vi "FRC Display Status Dialog.vi"(8 "error in":errorcluster, 9 "Numeric":u8, 10 "Text":string, 11 "Mode":T1(ring)) -> (0 "error out":errorcluster)   [LabVIEW 2027]
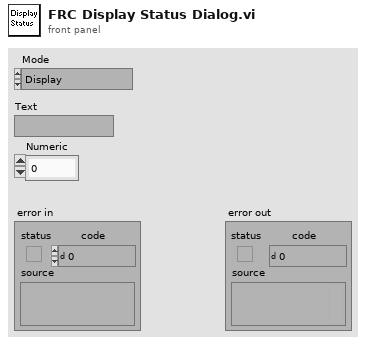
[diagram p1: front panel]
types:
  T1 = enum16{"Display", "Configure", "Hide Dialog", "Discard Ref"}
  T2 = enum32{"Invalid", "Standard", "Closed", "Hidden", "Minimized", "Maximized"}
  T3 = cluster{"Quit":bool, "Message":string, "Numeric":u8}
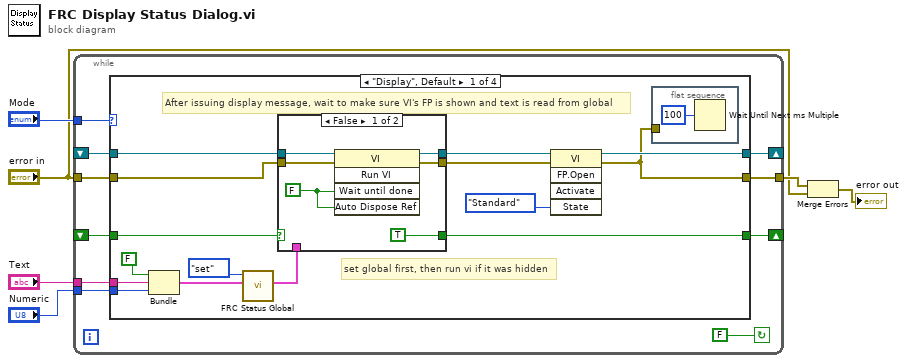
[diagram p0: block diagram]
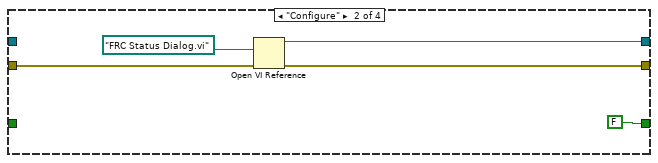
[diagram p3: hidden frame]
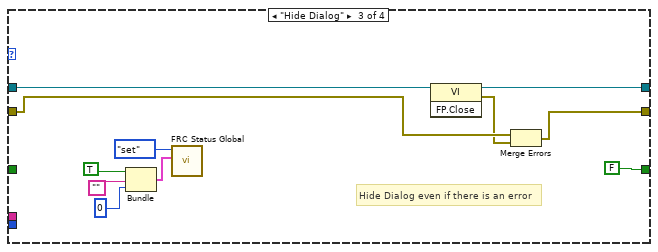
[diagram p4: hidden frame]
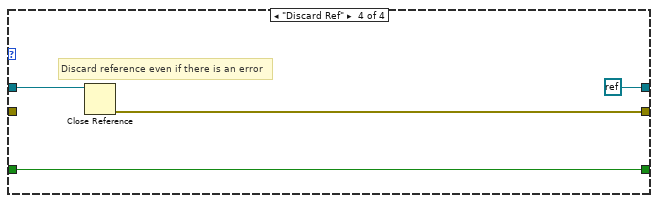
[diagram p5: hidden frame]
diagram:
  n1 = while {
    tunnel: "Mode" -> [w16]
    tunnel: "Text" -> [w14]
    shift-right: [w13] -> _
    shift-left: _ -> [w12]
    shift-right: [w10] -> _
    shift-left: _ -> [w11]
    tunnel: [w9] -> w3
    tunnel: "error in" -> [w8]
    tunnel: "Numeric" -> [w7]
    stop <- FALSE continue-if-true
    n2 = case shown="\"Display\", Default" w16 {
      tunnel: w14 -> [w27 _ _ _]
      tunnel: [w30 w46 w51 refnum<k0> refnum] -> w13
      tunnel: w12 -> [w31 _ w50 w59]
      tunnel: w11 -> [w29 _ _ w61]
      tunnel: [w28 FALSE FALSE w61] -> w10
      tunnel: [w18 w45 w47 w60] -> w9
      tunnel: w8 -> [w26 w44 w49 _]
      tunnel: w7 -> [w22 _ _ _]
      frame "Display", Default {
        # "After issuing display message, wait to make sure VI's FP is shown and text is read from global"
        # "set global first, then run vi if it was hidden"
        n3 = Bundle(FALSE, "Text"=w27, "Numeric"=w22) -> (w19:cluster{bool, "Text":string, "Numeric":u8})  [unwired: 1 out]
        n4 = call <resource>:"FRC Status Global.vi"("Data In"=w19, "Mode"=enum16{"get", "set"}."set" ("Switch")) -> ("Data Out"=w20:T3)  [unwired: 3 in, 6 out]
        n5 = case shown="False" w29 {
          selector: w29 -> [_ w40]
          tunnel: w31 -> [w38 w41]
          tunnel: [w37 w41] -> w25
          tunnel: [TRUE w40] -> w28
          tunnel: w26 -> [w34 w39]
          tunnel: [w35 w39] -> w24
          tunnel: w20 -> [_ _]
          frame False {
            w33 = FALSE ("Wait until done")
            n6 = invoke class="VI" method="Run VI"(reference=w38, error in=w34, "Wait until done"=w33, "Auto Dispose Ref"=w33) -> (reference out=w37:refnum<vi>, error out=w35:errorcluster)  [unwired: 1 in, 3 out]
          }
          frame True {
          }
        }
        n7 = invoke class="VI" method="FP.Open"(reference=w25, error in=w24, "State"=T2."Standard") -> (reference out=w30:refnum<vi>, error out=w18:errorcluster)  [unwired: 2 in, 3 out]
        n8 = flat-sequence {
          tunnel: w18 -> [_]
          frame #0 {
            n9 = Wait Until Next ms Multiple(millisecond multiple=u32 100) -> ()  [unwired: 1 out]
          }
        }
      }
      frame "Configure" {
        n10 = Open VI Reference(vi path=path "FRC Status Dialog.vi", error in (no error)=w44) -> (vi reference=w46:refnum<vi>, error out=w45:errorcluster)  [unwired: 4 out]
      }
      frame "Hide Dialog" {
        # "Hide Dialog even if there is an error"
        n11 = Bundle(TRUE, "", 0) -> (w52:cluster{bool, string, i32})  [unwired: 1 out]
        n12 = call <resource>:"FRC Status Global.vi"("Data In"=w52, "Mode"=enum16{"get", "set"}."set" ("Switch")) -> ()  [unwired: 3 in, 7 out]
        n13 = invoke class="VI" method="FP.Close"(reference=w50) -> (reference out=w51:refnum<vi>, error out=w48:errorcluster)  [unwired: 2 in, 1 out]
        n14 = Merge Errors(w49, w48) -> (w47:errorcluster)
      }
      frame "Discard Ref" {
        # "Discard reference even if there is an error"
        n15 = Close Reference(reference=w59) -> (error out=w60:errorcluster)  [unwired: 1 in]
      }
    }
  }
  n16 = Merge Errors(w3, "error in") -> (→"error out":errorcluster)
